vi "Analog_to_PWM_Ex.vi"() -> ()   [LabVIEW 2026]
panel:
  in  "Tab Control":enum32{"Read", "Write"}(tab)
  out "Waveform Chart 2":i32(graph)
  out "Square":dynamicdata(graph)
  in  "VISA resource name":refnum<visa-resource-name>
  in  "Stop Button":bool
  in  "Canal Read":u8
  in  "Canal Write":u8
  out "error out":errorcluster
  # "Ejemplo: Analog to PWM"
  # "Descripción: Convierte la lectura de un pin analógico en el ciclo de trabajo de una salida PWM."
  # "Configuracion"
  # "Indicadores"
  # "Control"
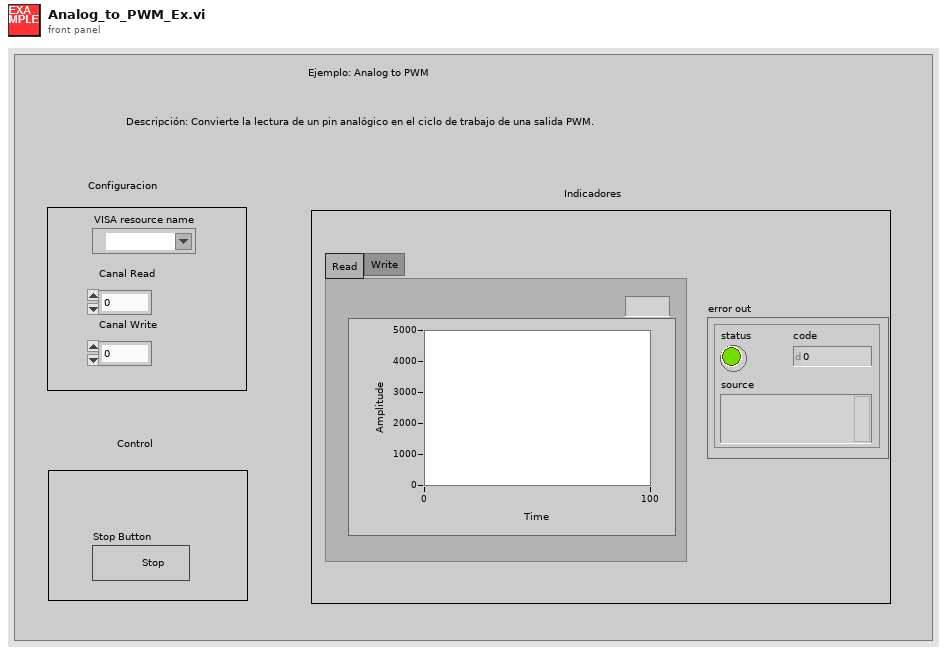
[diagram p1: front panel]
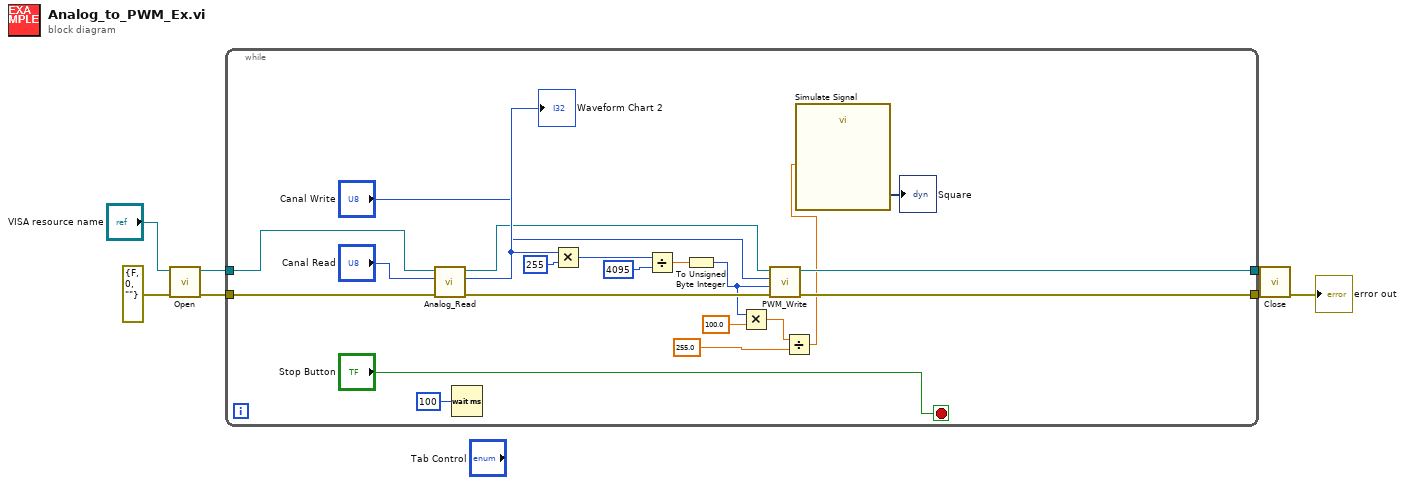
[diagram p0: block diagram]
diagram:
  n1 = call "Open.vi"("error in (no error)"=errorcluster {"status"=FALSE, "code"=0, "source"=""}, "VISA resource name"="VISA resource name") -> ("error out"=w7:errorcluster, "VISA resource name out"=w6:refnum<visa-resource-name>)  [unwired: 8 in]
  n2 = while {
    tunnel: w6 -> [w27]
    tunnel: w7 -> [w26]
    tunnel: [w18] -> w2
    tunnel: [w17] -> w1
    stop <- "Stop Button" stop-if-true
    n3 = call "Analog_Read.vi"("error in (no error)"=w26, "Canal"="Canal Read", "VISA resource name"=w27) -> ("error out"=w15:errorcluster, "Out"=w20:i32, "VISA resource name out"=w16:refnum<visa-resource-name>)  [unwired: 6 in]
    "Waveform Chart 2" <- w20
    n4 = Wait (ms)(milliseconds to wait=u32 100) -> ()  [unwired: 1 out]
    n5 = Multiply(x=w20, y=255) -> (x*y=w23:i32)
    n6 = Divide(x=w23, y=4095) -> (x/y=w21:dbl)
    n7 = To Unsigned Byte Integer(number=w21) -> (unsigned 8bit integer=w13:u8)
    n8 = Multiply(x=w13, y=100.0) -> (x*y=w11:dbl)
    n9 = call "PWM_Write.vi"("error in (no error)"=w15, "Duty Cycle"=w13, "Canal"="Canal Write", "VISA resource name"=w16) -> ("error out"=w17:errorcluster, "VISA resource name out"=w18:refnum<visa-resource-name>)  [unwired: 5 in, 1 out]
    n10 = Divide(x=w11, y=255.0) -> (x/y=w9:dbl)
    n11 = call "Simulate Signal"("Duty Cycle (%)"=w9) -> ("Square"=→"Square":dynamicdata)  [unwired: 13 in, 1 out]
  }
  n12 = call "Close.vi"("error in (no error)"=w1, "VISA resource name"=w2) -> ("error out"=→"error out":errorcluster)  [unwired: 9 in]
